vi "I2C Write Reg 16.vi"(8 "error in (no error)":errorcluster, 9 "Value":u16, 10 "Register":i32, 11 "I2C Device":T1) -> (0 "error out":errorcluster, 3 "I2C Device out":T1)   [LabVIEW 2020, in "wiringPi.lvlib"]
doc: "<b>_______________________________________________________________</b>\n** Author: Juan José Villacorta\n** LabVIEW wrapper for C library <b> wiringPi </b>,\n** https://github.com/WiringPi/WiringPi\n<b>_______________________________________________________________</b>\n/*\n * Write an 16-bit value to a register on the device\n**********************************************************************************\n*/"
uses:
  wiringPi.lvlib
  Type Defs/I2C Device.ctl
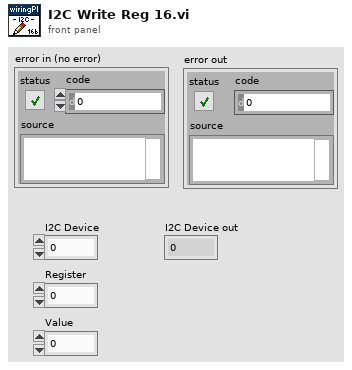
[diagram p1: front panel]
types:
  T1 = typedef "wiringPi.lvlib/I2C Device.ctl" = i32
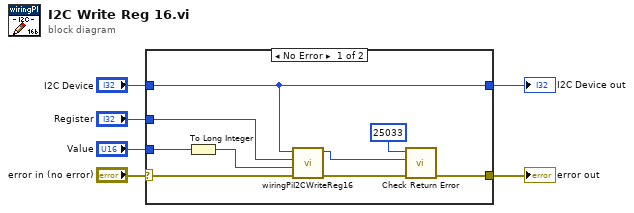
[diagram p0: block diagram]
diagram:
  n1 = case shown="No Error" "error in (no error)" {
    selector: "error in (no error)" -> [w14 w17]
    tunnel: [w15 w17] -> w5
    tunnel: "I2C Device" -> [w12 w16]
    tunnel: [w12 w16] -> w4
    tunnel: "Register" -> [w9 _]
    tunnel: "Value" -> [w8 _]
    frame No Error {
      n2 = To Long Integer(number=w8) -> (32bit integer=w7:i32)
      n3 = call "wiringPiI2CWriteReg16.vi"("error in (no error)"=w14, "value"=w7, "reg"=w9, "devID"=w12) -> ("error out"=w13:errorcluster, "return"=w11:i32)  [unwired: 6 in]
      n4 = call "Check Return Error.vi"("error in (no error)"=w13, "Return code"=w11, "Error number"=25033) -> ("error out"=w15:errorcluster)  [unwired: 8 in]
    }
    frame Error {
    }
  }
  "error out" <- w5
  "I2C Device out" <- w4
